vi "demo.vi"() -> ()   [LabVIEW 2016]
uses:
  main/apis/Setup/GetVI/GetVIByPath.vi
  main/apis/Stimulus/ValueSignalByPathString.vi
  <vilib>/addons/_JKI Toolkits/Caraya/classes/Test/Test.lvclass
panel:
  out "error out":errorcluster
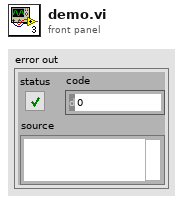
[diagram p1: front panel]
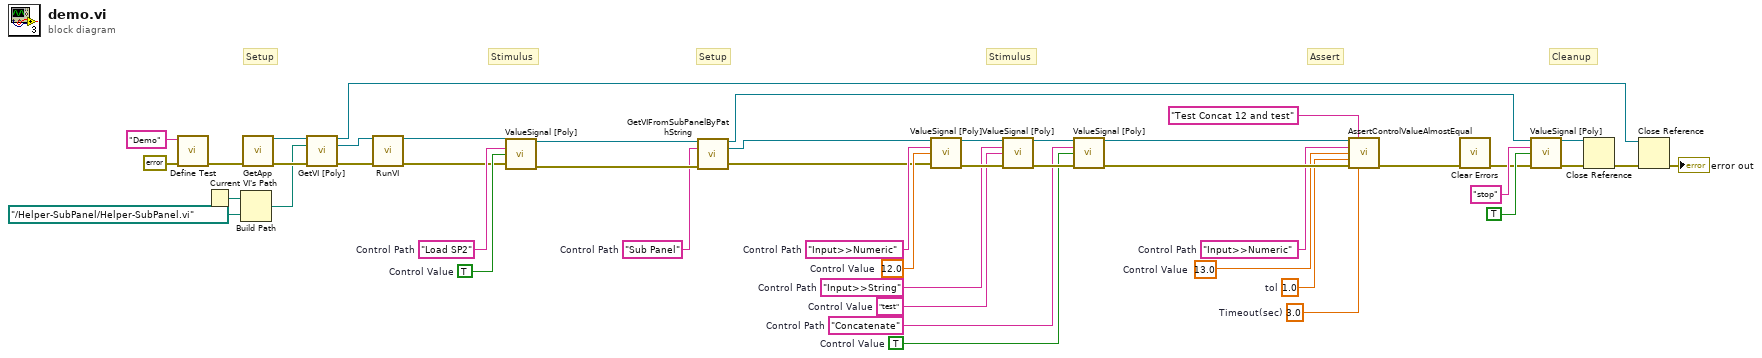
[diagram p0: block diagram]
diagram:
  w1 = 3.0  # Timeout(sec)
  w3 = 13.0  # Control Value
  w21 = "Input>>String"  # Control Path
  w22 = "Sub Panel"  # Control Path
  w2 = 1.0  # tol
  w4 = "Input>>Numeric"  # Control Path
  w27 = "Input>>Numeric"  # Control Path
  w28 = TRUE  # Control Value
  w29 = "Concatenate"  # Control Path
  w32 = "test"  # Control Value
  w35 = 12.0  # Control Value
  w36 = TRUE  # Control Value
  w37 = "Load SP2"  # Control Path
  # "Cleanup"
  # "Assert"
  # "Setup"
  # "Stimulus"
  # "Stimulus"
  # "Setup"
  n1 = call <vilib>:"Define Test.vi"("error in (no error)"=errorcluster {"status"=FALSE, "code"=0, "source"=""}, "Label (VI Title)"="Demo") -> ("error out"=w45:errorcluster)  [unwired: 9 in]
  n2 = Current VI's Path() -> (path=w17:path)
  n3 = Build Path(base path=w17, name or relative path=path "../Helper-SubPanel/Helper-SubPanel.vi" ("path")) -> (appended path=w18:path)
  n4 = call "GetApp.vi"("error in (no error)"=w45) -> ("Application Ref"=w43:refnum<vi>, "error out"=w42:errorcluster)  [unwired: 13 in]
  n5 = call-poly "GetVI [Poly].vi"("Application Ref in"=w43, "VI Path"=w18, "error in (no error)"=w42) -> ("Application Ref out"=w41:refnum<vi>, "VI Reference"=w13:refnum<vi>, "error out"=w15:errorcluster)  [unwired: 10 in]
  n6 = call "RunVI.vi"("VI Reference In"=w13, "error in"=w15) -> ("VI Reference Out"=w12:refnum<vi>, "error out"=w14:errorcluster)  [unwired: 12 in]
  n7 = call-poly "ValueSignal [Poly].vi"("VI Reference In"=w12, "Control Name"=w37, "Value (Signaling)"=w36, "error in"=w14) -> ("VI Reference Out"=w25:refnum<vi>, "error out"=w26:errorcluster)  [unwired: 10 in]
  n8 = call "GetVIFromSubPanelByPathString.vi"("VI Reference In"=w25, "SubPanel Path"=w22, "error in"=w26) -> ("VI Reference Out"=w20:refnum<vi>, "SubPanel VI Reference"=w23:refnum<vi>, "error out"=w24:errorcluster)  [unwired: 10 in]
  n9 = call-poly "ValueSignal [Poly].vi"("VI Reference In"=w23, "Control Name"=w27, "Value (Signaling)"=w35, "error in"=w24) -> ("VI Reference Out"=w33:refnum<vi>, "error out"=w34:errorcluster)  [unwired: 10 in]
  n10 = call-poly "ValueSignal [Poly].vi"("VI Reference In"=w33, "Control Name"=w21, "Value (Signaling)"=w32, "error in"=w34) -> ("VI Reference Out"=w30:refnum<vi>, "error out"=w31:errorcluster)  [unwired: 10 in]
  n11 = call-poly "ValueSignal [Poly].vi"("VI Reference In"=w30, "Control Name"=w29, "Value (Signaling)"=w28, "error in"=w31) -> ("VI Reference Out"=w5:refnum<vi>, "error out"=w8:errorcluster)  [unwired: 10 in]
  n12 = call "AssertControlValueAlmostEqual.vi"("VI Reference In"=w5, "Label"="Test Concat 12 and test", "Control Name"=w4, "Control Value"=w3, "Tolerance"=w2, "error out"=w8, "Timeout(5 sec)"=w1) -> ("error out"=w7:errorcluster)  [unwired: 7 in, 1 out]
  n13 = call <vilib>:"Clear Errors.vi"("error in (no error)"=w7) -> ("error out"=w9:errorcluster)  [unwired: 5 in, 1 out]
  n14 = call-poly "ValueSignal [Poly].vi"("VI Reference In"=w20, "Control Name"="stop" ("Class Name"), "Value (Signaling)"=TRUE, "error in"=w9) -> ("VI Reference Out"=w38:refnum<vi>, "error out"=w39:errorcluster)  [unwired: 10 in]
  n15 = Close Reference(reference=w38, error in (no error)=w39) -> (error out=w40:errorcluster)
  n16 = Close Reference(reference=w41, error in (no error)=w40) -> (error out=→"error out":errorcluster)
